vi "Configure_DAC_Source.vi"(0 "IVI Refnum in":refnum<k15>, 1 "Source Mode":T2 caption="source mode" items=["Single Point"=1020, "Sequence"=1021], 5 "Current Limit":dbl, 7 "Voltage Level Range":dbl, 11 "Error In":errorcluster, 12 "Output Function":T1 caption="output function" items=["DC Voltage"=1006, "DC Current"=1007, "Pulse Voltage"=1049, "Pulse Current"=1050, "Constant Resistance"=1161, "Constant Power"=1162]) -> (4 "Instrument Handle":refnum<k15> caption="instrument handle out", 15 "Error Out":errorcluster)   [LabVIEW 2026, in "Core.lvlib"]
uses:
  Core.lvlib
  <instrlib>/niDCPower/nidcpower.llb/niDCPower Source Mode.ctl
  <instrlib>/niDCPower/nidcpower.llb/niDCPower Output Function.ctl
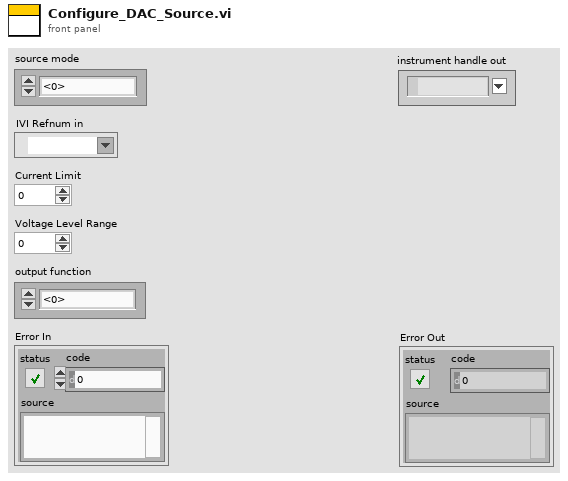
[diagram p1: front panel]
types:
  T1 = typedef "niDCPower Output Function.ctl" = i32
  T2 = typedef "niDCPower Source Mode.ctl" = i32
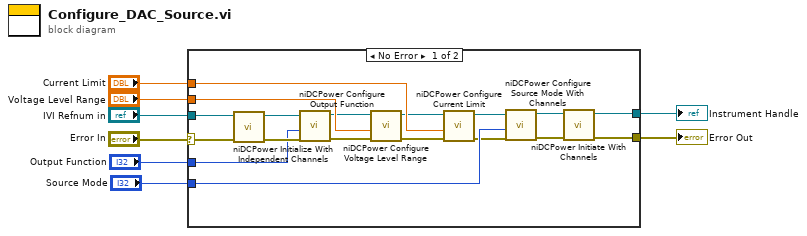
[diagram p0: block diagram]
diagram:
  n1 = case shown="No Error" "Error In" {
    selector: "Error In" -> [w26 w27]
    tunnel: "Source Mode" -> [w22 _]
    tunnel: "Current Limit" -> [w20 _]
    tunnel: "Voltage Level Range" -> [w19 _]
    tunnel: "IVI Refnum in" -> [w18 w28]
    tunnel: "Output Function" -> [w11 _]
    tunnel: [w10 w27] -> w2
    tunnel: [w9 w28] -> w1
    frame No Error {
      n2 = call <instrlib>:"niDCPower Initialize With Independent Channels.vi"("error in (no error)"=w26, "resource name"=w18) -> ("error out"=w13:errorcluster, "instrument handle out"=w12:refnum<k15>)  [unwired: 8 in]
      n3 = call <instrlib>:"niDCPower Configure Output Function.vi"("error in (no error)"=w13, "output function"=w11, "instrument handle"=w12) -> ("error out"=w14:errorcluster, "instrument handle out"=w16:refnum<k15>)  [unwired: 7 in]
      n4 = call <instrlib>:"niDCPower Configure Voltage Level Range.vi"("error in (no error)"=w14, "voltage level range"=w19, "instrument handle"=w16) -> ("error out"=w15:errorcluster, "instrument handle out"=w17:refnum<k15>)  [unwired: 7 in]
      n5 = call <instrlib>:"niDCPower Configure Current Limit.vi"("error in (no error)"=w15, "current limit"=w20, "instrument handle"=w17) -> ("error out"=w21:errorcluster, "instrument handle out"=w23:refnum<k15>)  [unwired: 7 in]
      n6 = call <instrlib>:"niDCPower Configure Source Mode With Channels.vi"("error in (no error)"=w21, "source mode"=w22, "instrument handle"=w23) -> ("error out"=w24:errorcluster, "instrument handle out"=w25:refnum<k15>)  [unwired: 7 in]
      n7 = call <instrlib>:"niDCPower Initiate With Channels.vi"("error in (no error)"=w24, "instrument handle"=w25) -> ("error out"=w10:errorcluster, "instrument handle out"=w9:refnum<k15>)  [unwired: 8 in]
    }
    frame Error {
    }
  }
  "Error Out" <- w2
  "Instrument Handle" <- w1
